vi "Game_Place_Stone.vi"(0 "Board State":T3={"Grid"=array15x15[225 elements], "Move History"=[], "Last Move"={"Row"=-1, "Col"=-1, "Stone"=enum."Empty"}}, 5 "Move":T4={"Row"=7, "Col"=7, "Stone"=enum."Black"}, 7 "Renju":bool=TRUE, 11 "error in":errorcluster) -> (3 "Draw?":bool, 4 "Board State out":T3={"Grid"=array15x15[225 elements], "Move History"=[], "Last Move"={"Row"=-1, "Col"=-1, "Stone"=enum."Empty"}}, 6 "Placed?":bool, 8 "Win?":bool, 10 "Win Line":T2(array[cluster]), 14 "Forbidden Reason":T1(ring), 15 "error out":errorcluster)   [LabVIEW 2026]
doc: "착수 처리: 범위/빈 칸/렌주 금수 검사 후 Grid, Move History, Last Move 갱신, 승리/무승부 판정.\nPlaced?=False면 Board State는 그대로, Forbidden Reason에 금수 사유."
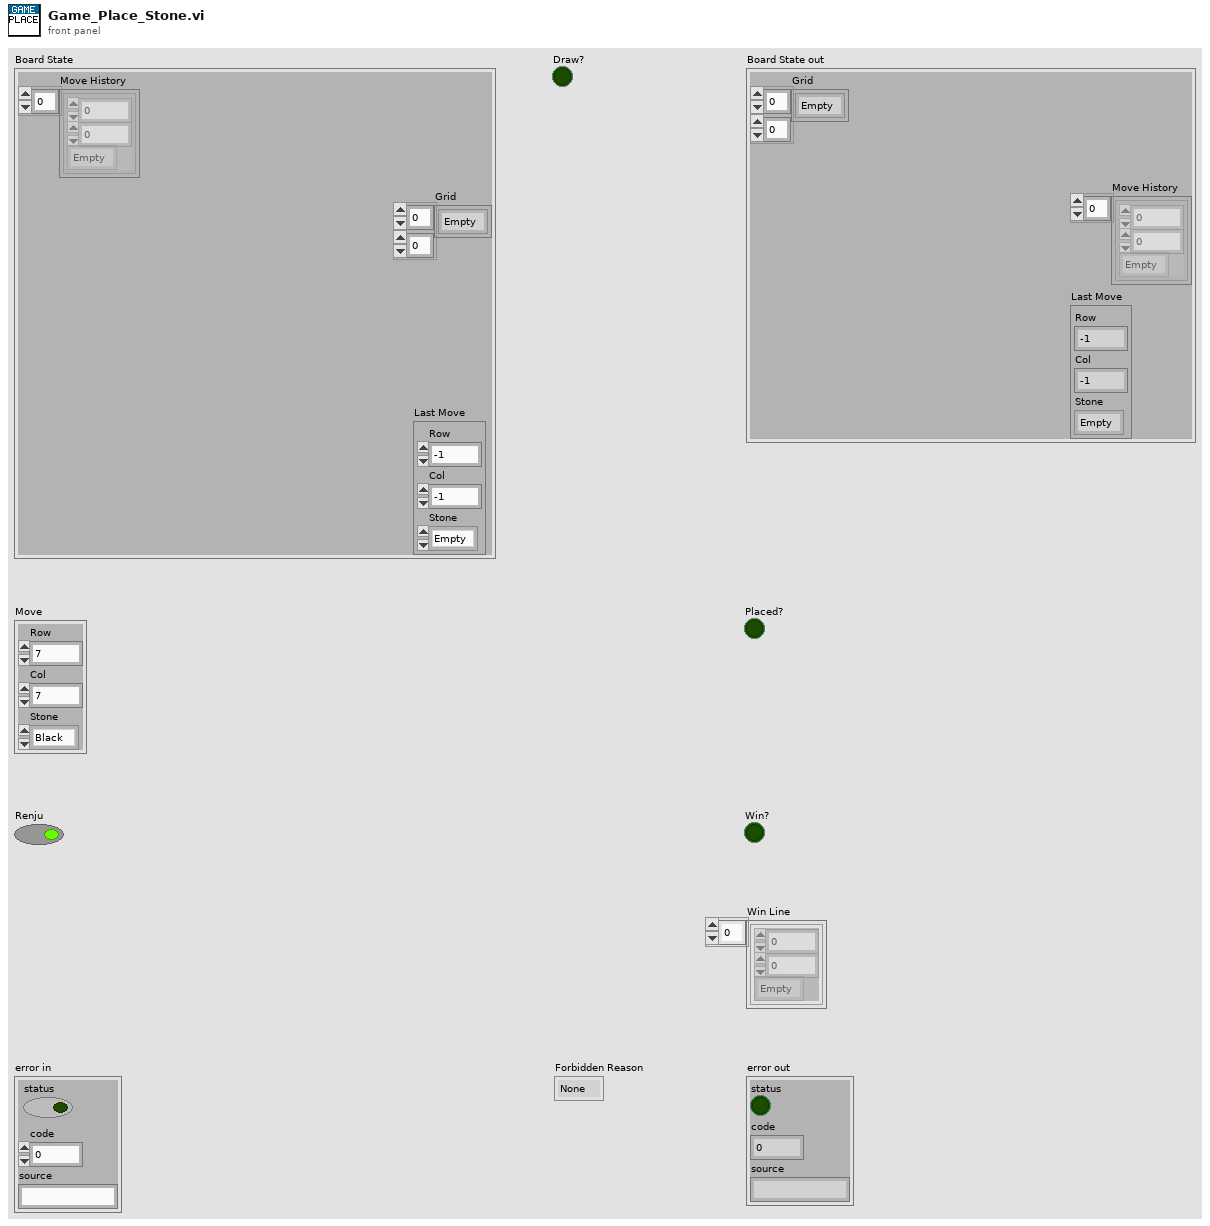
[diagram p1: front panel]
types:
  T1 = enum8{"None", "Double Three", "Double Four", "Overline"}
  T2 = cluster{"Row":i32, "Col":i32, "Stone":enum8{"Empty", "Black", "White"}}[]
  T3 = cluster{"Grid":enum8{"Empty", "Black", "White"}[][], "Move History":cluster{"Row":i32, "Col":i32, "Stone":enum8{"Empty", "Black", "White"}}[], "Last Move":cluster{"Row":i32, "Col":i32, "Stone":enum8{"Empty", "Black", "White"}}}
  T4 = cluster{"Row":i32, "Col":i32, "Stone":enum8{"Empty", "Black", "White"}}
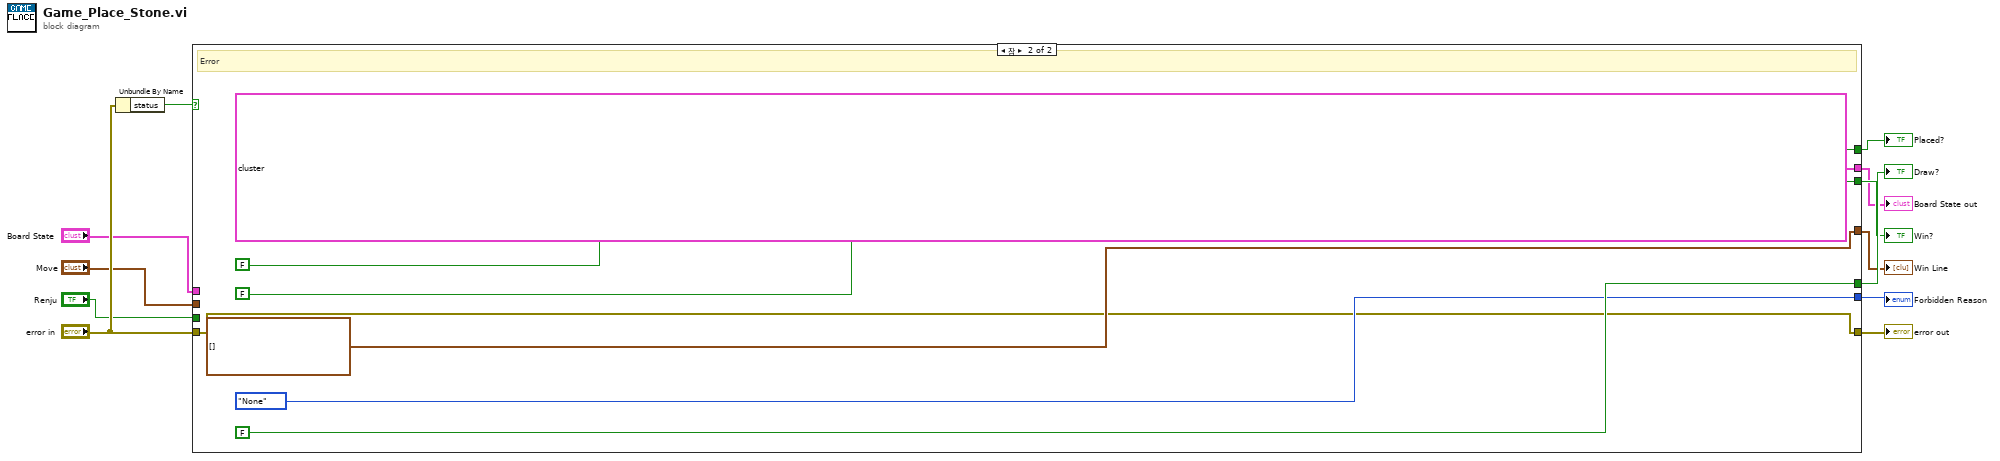
[diagram p0: block diagram]
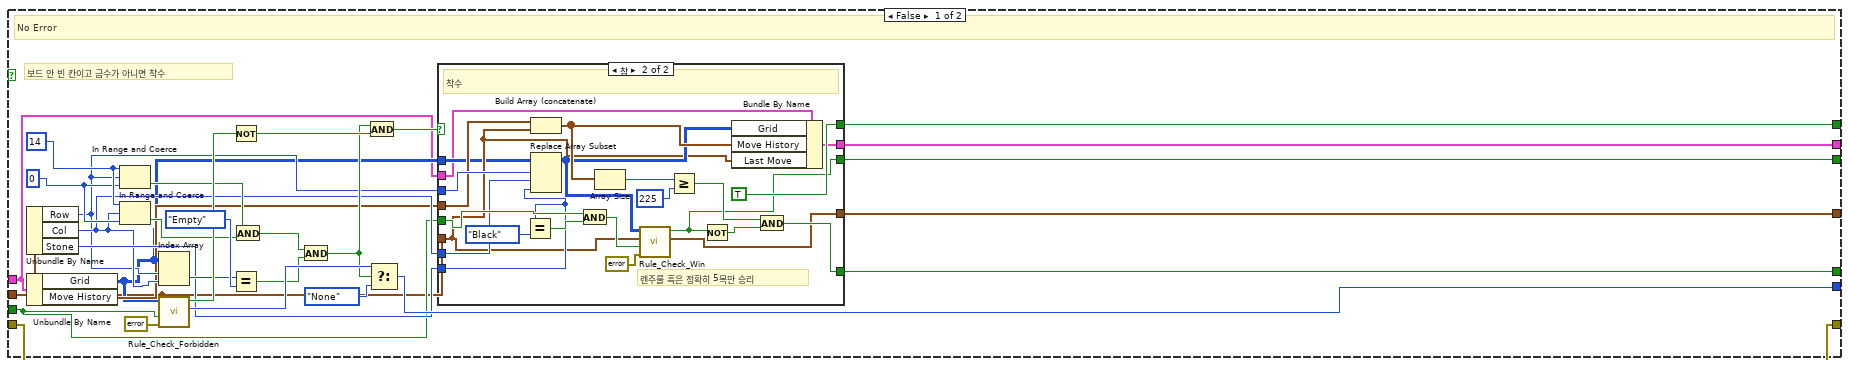
[diagram p2: hidden frame]
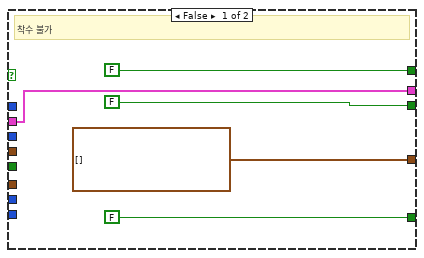
[diagram p3: hidden frame]
diagram:
  n1 = Unbundle By Name("error in") -> ("status"=w5:bool)
  n2 = case shown="참" w5 {
    tunnel: "Board State" -> [w13 _]
    tunnel: "Move" -> [w14 _]
    tunnel: "Renju" -> [w15 _]
    tunnel: "error in" -> [w16 w71]
    tunnel: [w37 FALSE] -> w7
    tunnel: [w16 w71] -> w12
    tunnel: [w36 T3 {"Grid"=array15x15[225 elements], "Move History"=[], "Last Move"={"Row"=-1, "Col"=-1, "Stone"=enum."Empty"}}] -> w6
    tunnel: [w42 T1."None"] -> w10
    tunnel: [w38 FALSE] -> w8
    tunnel: [w39 T2 []] -> w9
    tunnel: [w40 FALSE] -> w11
    frame False {
      w23 = 14
      w22 = 0
      # "보드 안 빈 칸이고 금수가 아니면 착수"
      # "No Error"
      n3 = Unbundle By Name(w14) -> ("Row"=w19:i32, "Col"=w20:i32, "Stone"=w21:enum8{"Empty", "Black", "White"})
      n4 = Unbundle By Name(w13) -> ("Grid"=w17:enum8{"Empty", "Black", "White"}[][], "Move History"=w18:T2)
      n5 = In Range and Coerce(upper limit=w23, x=w19, lower limit=w22) -> (In Range?=w24:bool)  [unwired: 1 out]
      n6 = In Range and Coerce(upper limit=w23, x=w20, lower limit=w22) -> (In Range?=w25:bool)  [unwired: 1 out]
      n7 = Index Array(array=w17, index (row)=w19, index (col)=w20) -> (element=w27:enum8{"Empty", "Black", "White"})
      n8 = call "Rule_Check_Forbidden.vi"("error in"=errorcluster {"status"=FALSE, "code"=0, "source"=""}, "Renju"=w15, "Move"=w14, "Grid"=w17) -> ("Reason"=w33:T1, "Forbidden?"=w32:bool)  [unwired: 5 in, 1 out]
      n9 = Not(x=w32) -> (.not. x?=w34:bool)
      n10 = Equal?(x=w27, y=enum8{"Empty", "Black", "White"}."Empty") -> (x = y?=w29:bool)
      n11 = And(x=w24, y=w25) -> (x .and. y?=w26:bool)
      n12 = And(x=w26, y=w29) -> (x .and. y?=w30:bool)
      n13 = And(x=w30, y=w34) -> (x .and. y?=w35:bool)
      n14 = Select(t=w33, s=w30, f=T1."None") -> (s? t:f=w42:T1)
      n15 = case shown="참" w35 {
        tunnel: [FALSE TRUE] -> w37
        tunnel: w13 -> [w43 w48]
        tunnel: w14 -> [_ w51]
        tunnel: w15 -> [_ w55]
        tunnel: w17 -> [_ w49]
        tunnel: w18 -> [_ w50]
        tunnel: w19 -> [_ w52]
        tunnel: w20 -> [_ w53]
        tunnel: w21 -> [_ w54]
        tunnel: [w43 w58] -> w36
        tunnel: [FALSE w63] -> w38
        tunnel: [T2 [] w64] -> w39
        tunnel: [FALSE w69] -> w40
        frame False {
          # "착수 불가"
        }
        frame True {
          # "렌주룰 흑은 정확히 5목만 승리"
          # "착수"
          n16 = Equal?(x=w54, y=enum8{"Empty", "Black", "White"}."Black") -> (x = y?=w60:bool)
          n17 = Build Array (concatenate)(w50, w51) -> (w57:T2)
          n18 = Replace Array Subset(array=w49, new element=w54, index (row)=w52, index (col)=w53) -> (w56:enum8{"Empty", "Black", "White"}[][])
          n19 = And(x=w55, y=w60) -> (x .and. y?=w61:bool)
          n20 = Array Size(array=w57) -> (size(s)=w65:i32)
          n21 = call "Rule_Check_Win.vi"("error in"=errorcluster {"status"=FALSE, "code"=0, "source"=""}, "Exact Five"=w61, "Last Move"=w51, "Grid"=w56) -> ("Win Line"=w64:T2, "Win?"=w63:bool)  [unwired: 4 in, 2 out]
          n22 = Greater Or Equal?(x=w65, y=225) -> (x >= y?=w67:bool)
          n23 = Not(x=w63) -> (.not. x?=w68:bool)
          n24 = Bundle By Name(cluster=w48, "Grid"=w56, "Move History"=w57, "Last Move"=w51) -> (w58:T3)
          n25 = And(x=w67, y=w68) -> (x .and. y?=w69:bool)
        }
      }
    }
    frame True {
      # "Error"
    }
  }
  "Board State out" <- w6
  "Placed?" <- w7
  "Win?" <- w8
  "Win Line" <- w9
  "Forbidden Reason" <- w10
  "Draw?" <- w11
  "error out" <- w12
